vi "RemoteVI Server Windows.vi"(0 "labview only?":bool, 1 "skip":u64, 2 "selected hWnd":u64) -> (4 "rows":T1(array[cluster]), 5 "items":string[][](array[string]), 6 "selected":i32=-1)   [LabVIEW 2020, in "RemoteVI.lvlib"]
doc: "The list of RemoteVI Server: the shareable windows (RemoteVI List Top Windows.vi, then RemoteVI Window Rows.vi - LabVIEW first, then LabVIEW-built applications, then other programs) and their listbox rows window | program | kind. selected is the row of the window selected hWnd in the new list (-1 when it is gone), so the selection follows the window when the list changes."
uses:
  RemoteVI.lvlib
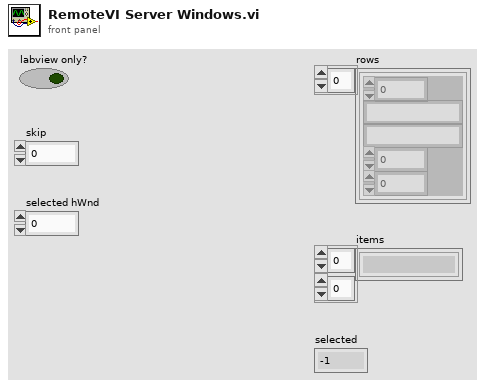
[diagram p1: front panel]
types:
  T1 = cluster{"group":i32, "program":string, "title":string, "pid":u32, "hWnd":u64}[]
  T2 = cluster{"hWnd":u64, "pid":u32, "path":string, "class":string, "title":string, "visible":bool, "owned":bool, "ex style":u32, "w":i32, "h":i32}[]
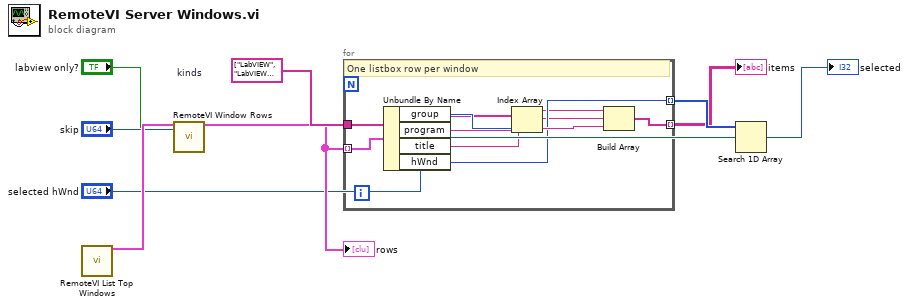
[diagram p0: block diagram]
diagram:
  w6 = string[] ["LabVIEW", "LabVIEW app", "Other program"]  # kinds
  n1 = call "RemoteVI List Top Windows.vi"() -> ("windows"=w4:T2)  [unwired: 15 in]
  n2 = call "RemoteVI Window Rows.vi"("raw"=w4, "labview only?"="labview only?", "skip"="skip") -> ("rows"=w5:T1)  [unwired: 12 in]
  "rows" <- w5
  n3 = for {
    tunnel: w6 -> [w11]
    tunnel: w5 -> [w10] mode=indexing
    tunnel: [w15] -> w8 mode=indexing
    tunnel: [w17] -> w7 mode=indexing
    # "One listbox row per window"
    n4 = Unbundle By Name(w10) -> ("group"=w12:i32, "program"=w13:string, "title"=w14:string, "hWnd"=w15:u64)
    n5 = Index Array(array=w11, index=w12) -> (element=w16:string)
    n6 = Build Array(w14, w13, w16) -> (w17:string[])
  }
  "items" <- w7
  n7 = Search 1D Array(1D array=w8, element="selected hWnd") -> (index of element=→"selected":i32)  [unwired: 1 in]
